vi "Riccati_Check_Detectable.vi"(9 "Q":T1, 11 "A":T1) -> (0 "error out":errorcluster, 1 "Stable Bad":bool, 2 "Pos Semi Definite":bool, 3 "Bad":bool, 4 "Q_Check":T1, 5 "C":T1, 6 "Q_Chk_Passed":bool)   [LabVIEW 2019, in "Trajectory_Library.lvlib"]
doc: "This function is for internal use, by the riccati_iput_check, ONLY.\n\nThis function check if (A,C) is a detectable pair, where Q = C' * C. (A,C) is detectable if and only if the unobservable eigenvalues of A, if any, have absolute values less than one, where an eigenvalue is unobservable if Rank[lambda * I - A; C] < n. Also, (A,C) is detectable if and only if (A',C') is stabilizable.\n\nInputs:\n - A -- A matrix\n - Q -- Q matrix\n\nOutputs:\n - Bad -- Returns TRUE, if the A,Q pair is not detectable or an error occured.\n - Error -- Error cluster that returns an error if A, Q is not detectable or some other error occured."
uses:
  Trajectory_Library.lvlib
  <vilib>/Analysis/Matrix/Datatypes/RealMatrix.ctl
  <vilib>/Analysis/_algsub.llb/Matrix Type for Test.ctl
  <vilib>/Analysis/baseanly.llb/Real A x B.vi
  <vilib>/Analysis/7linalg.llb/Real LU Factorization.vi
  <vilib>/Analysis/Matrix/Numeric/Subtract/Subtract - RM,RM.vi
  <vilib>/Analysis/Matrix/Numeric/Absolute Value/Absolute Value - RM.vi
  <vilib>/Analysis/_algsub.llb/Test Real Matrix Type.vi
  <vilib>/Analysis/NI_AALBase.lvlib
  <vilib>/Analysis/NI_AALPro.lvlib
  <vilib>/Analysis/Matrix/NI_Matrix.lvlib
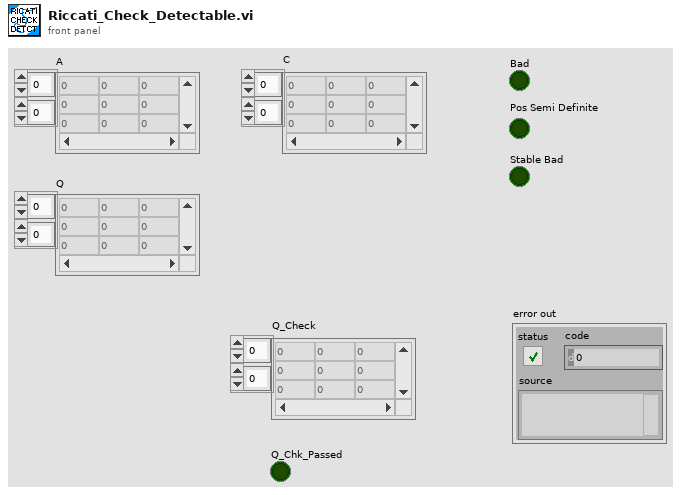
[diagram p1: front panel]
types:
  T1 = typedef "NI_Matrix.lvlib/RealMatrix.ctl" = dbl[][]
  T2 = typedef "NI_AALPro.lvlib/Matrix Type for Test.ctl" = i32
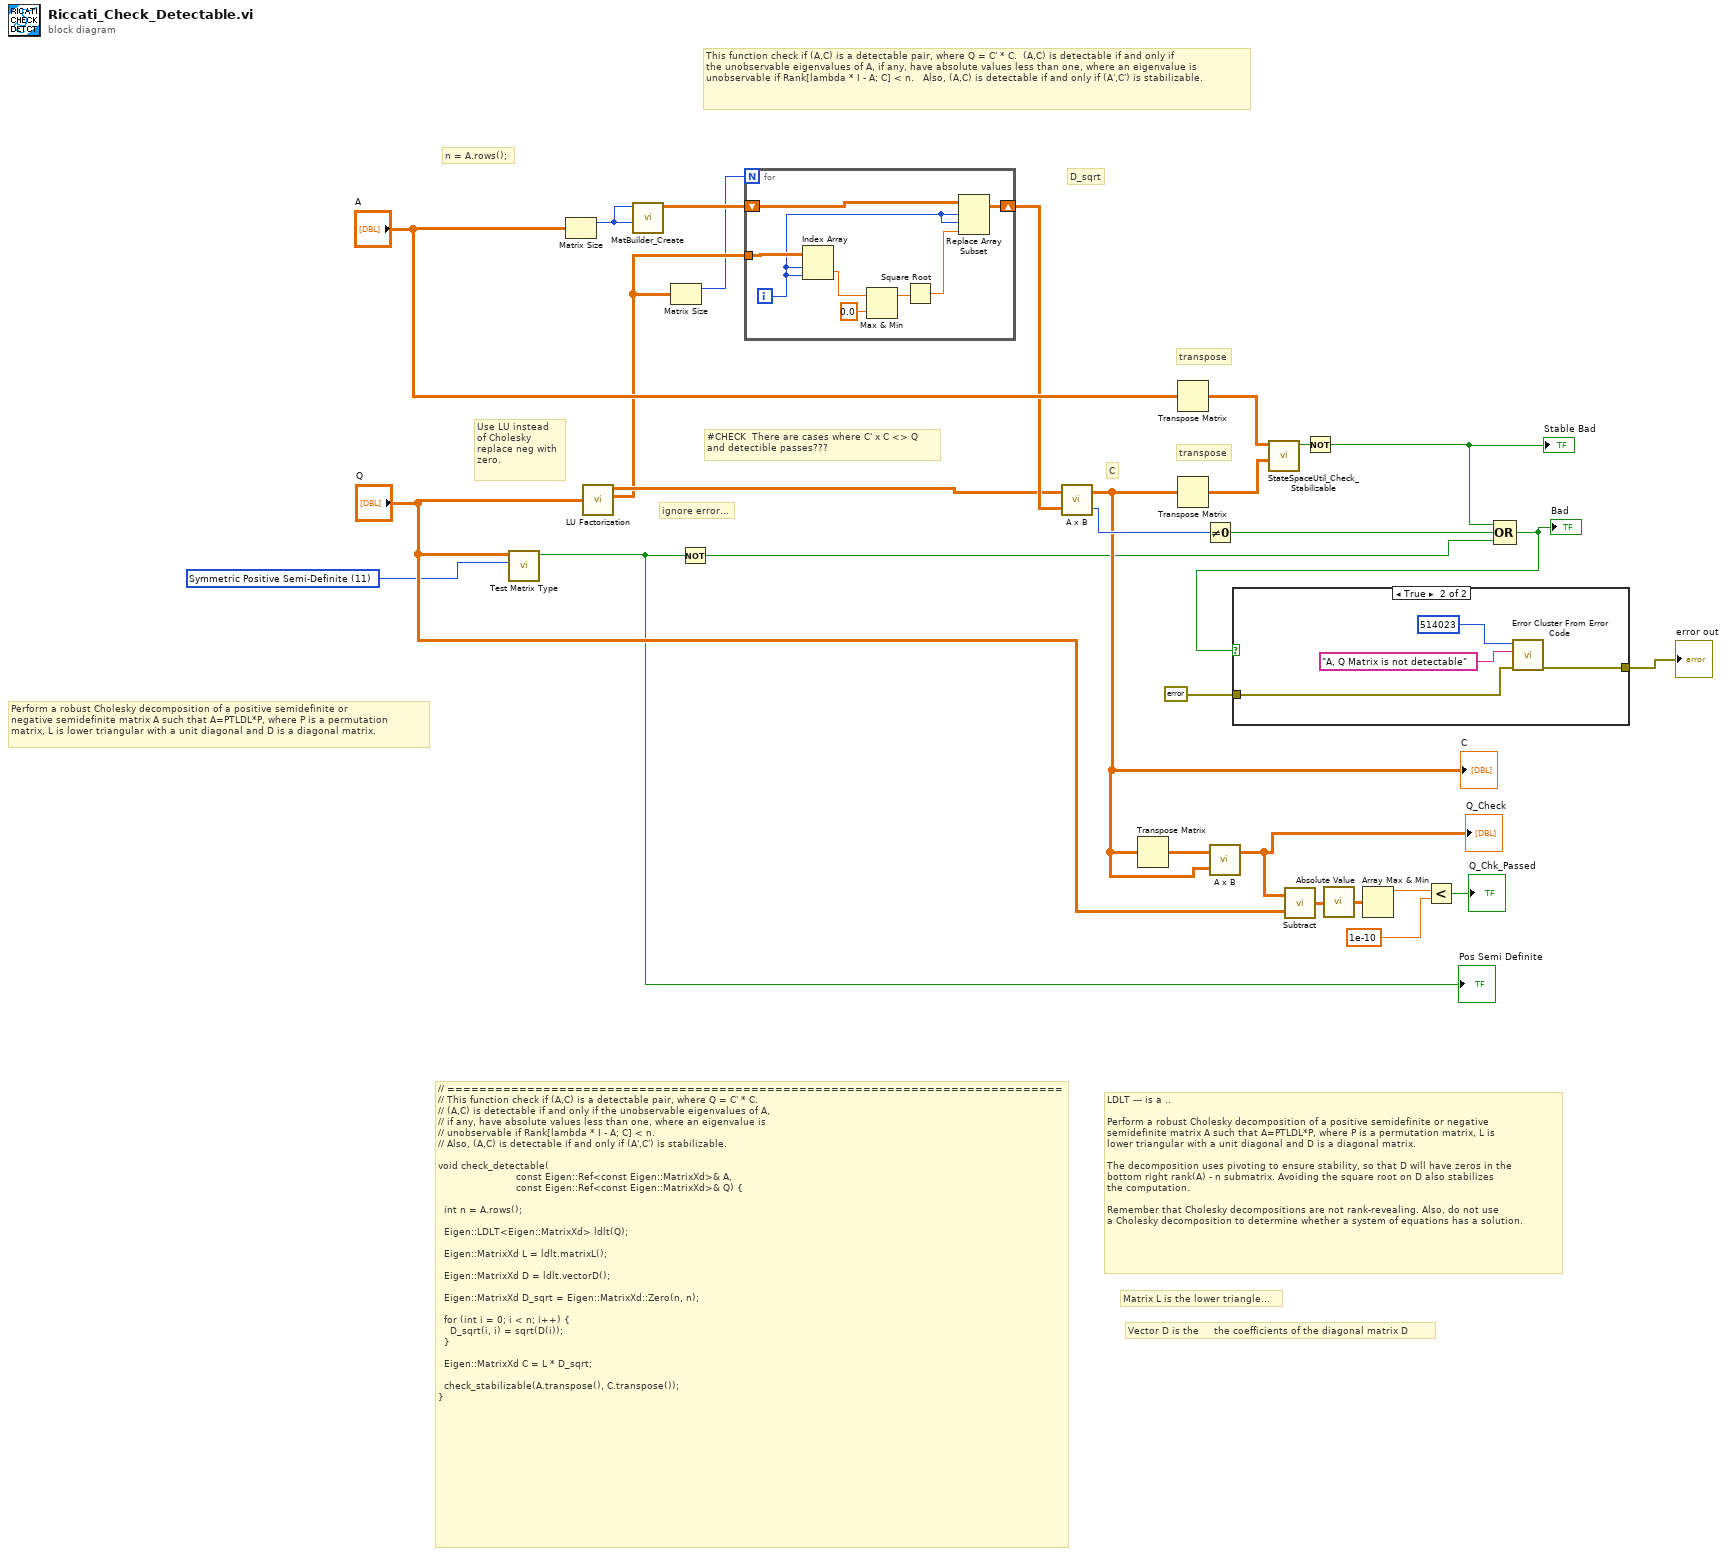
[diagram p0: block diagram]
diagram:
  w6 = T2 11 items=["Symmetric Positive Definite"=10, "Symmetric Positive Semi-Definite"=11, "Symmetric"=20, "Hermitian"=21] ("matrix type")
  # "#CHECK  There are cases where C' x C <> Q \nand detectible passes???"
  # "ignore error..."
  # "Use LU instead\nof Cholesky\nreplace neg with\nzero."
  # "C"
  # "Vector D is the     the coefficients of the diagonal matrix D"
  # "Matrix L is the lower triangle..."
  # "LDLT --- is a ..\n\nPerform a robust Cholesky decomposition of a positive semidefinite or negative \nsemidefinite matrix A such that A=PTLDL*P, where P is a permutation matrix, L is \nlower triangular with a unit diagonal and D is a diagonal matrix.\n\nThe decomposition uses pivoting to ensure stability, so that D will have zeros in the \nbottom right rank(A) - n submatrix. Avoiding the square root on D also stabilizes \nthe computation.\n\nRemember that Cholesky decompositions are not rank-revealing. Also, do not use \na Cholesky decomposition to determine whether a system of equations has a solution."
  # "This function check if (A,C) is a detectable pair, where Q = C' * C.  (A,C) is detectable if and only if \nthe unobservable eigenvalues of A, if any, have absolute values less than one, where an eigenvalue is \nunobservable if Rank[lambda * I - A; C] < n.   Also, (A,C) is detectable if and only if (A',C') is stabilizable."
  # "transpose"
  # "transpose"
  # "D_sqrt"
  # "Perform a robust Cholesky decomposition of a positive semidefinite or \nnegative semidefinite matrix A such that A=PTLDL*P, where P is a permutation \nmatrix, L is lower triangular with a unit diagonal and D is a diagonal matrix."
  # "n = A.rows();"
  # "// =============================================================================\n// This function check if (A,C) is a detectable pair, where Q = C' * C.\n// (A,C) is detectable if and only if the unobservable eigenvalues of A,\n// if any, have absolute values less than one, where an eigenvalue is\n// unobservable if Rank[lambda * I - A; C] < n.\n// Also, (A,C) is detectable if and only if (A',C') is stabilizable.\n\nvoid check_detectable(\n                          const Eigen::Ref<const Eigen::MatrixXd>& A,\n                          const Eigen::Ref<const Eigen::MatrixXd>& Q) {\n\n  int n = A.rows();\n\n  Eigen::LDLT<Eigen::MatrixXd> ldlt(Q);\n\n  Eigen::MatrixXd L = ldlt.matrixL();\n\n  Eigen::MatrixXd D = ldlt.vectorD();\n\n  Eigen::MatrixXd D_sqrt = Eigen::MatrixXd::Zero(n, n);\n\n  for (int i = 0; i < n; i++) {\n    D_sqrt(i, i) = sqrt(D(i));\n  }\n\n  Eigen::MatrixXd C = L * D_sqrt;\n\n  check_stabilizable(A.transpose(), C.transpose());\n}"
  n1 = call-poly <vilib>:"Test Matrix Type.vi"("matrix type"=w6, "Input Matrix"="Q") -> ("is type?"=w5:bool)  [unwired: 8 in, 1 out]
  "Pos Semi Definite" <- w5
  n2 = Matrix Size(0:"A") -> (1:w25:i32)  [unwired: 1 out]
  n3 = call-poly <vilib>:"LU Factorization.vi"("A"="Q") -> ("L"=w18:T1, "U"=w17:T1)  [unwired: 2 out]
  n4 = call "MatBuilder_Create.vi"("Columns"=w25, "Rows"=w25) -> ("output matrix"=w24:T1)  [unwired: 9 in]
  n5 = Matrix Size(0:w17) -> (1:w16:i32)  [unwired: 1 out]
  n6 = Not(x=w5) -> (.not. x?=w4:bool)
  n7 = for {
    N: w16 -> [_]
    tunnel: w17 -> [w36]
    shift-right: [w34] -> w22
    shift-left: w24 -> [w35]
    i -> [w29]
    n8 = Index Array(array=w36, index (row)=w29, index (col)=w29) -> (element=w32:dbl)
    n9 = Max & Min(x=w32, y=0.0) -> (max(x,y)=w30:dbl)  [unwired: 1 out]
    n10 = Square Root ("Square Root.vi")(x=w30) -> (sqrt(x)=w33:dbl)
    n11 = Replace Array Subset(array=w35, new element=w33, index (row)=w29, index (col)=w29) -> (w34:T1)
  }
  n12 = call-poly <vilib>:"A x B.vi"("B"=w22, "A"=w18) -> ("error"=w23:i32, "A x B"=w14:T1)
  "C" <- w14
  n13 = Transpose Matrix(1:w14) -> (0:w15:T1)
  n14 = Transpose Matrix(1:"A") -> (0:w28:T1)
  n15 = Transpose Matrix(1:w14) -> (0:w27:T1)
  n16 = Not Equal To 0?(x=w23) -> (x != 0?=w21:bool)
  n17 = call-poly <vilib>:"A x B.vi"("B"=w14, "A"=w15) -> ("A x B"=w13:T1)  [unwired: 1 out]
  "Q_Check" <- w13
  n18 = call "StateSpaceUtil_Check_Stabilizable.vi"("B"=w27, "A"=w28) -> ("IsStabilizable"=w20:bool)  [unwired: 6 in, 3 out]
  n19 = call-poly <vilib>:"Subtract.vi"("Real Matrix B"="Q", "Real Matrix A"=w13) -> ("A - B"=w12:T1)
  n20 = Not(x=w20) -> (.not. x?=w19:bool)
  "Stable Bad" <- w19
  n21 = call-poly <vilib>:"Absolute Value.vi"("Real Matrix A"=w12) -> ("|A|"=w11:T1)
  n22 = Array Max & Min(array=w11) -> (max value=w10:dbl)  [unwired: 3 out]
  n23 = Less?(x=w10, y=1e-10) -> (x < y?=→"Q_Chk_Passed":bool)
  n24 = Compound Arithmetic op=OR(w19, w21, w4) -> (w3:bool)
  "Bad" <- w3
  n25 = case shown="True" w3 {
    tunnel: errorcluster {"status"=FALSE, "code"=0, "source"=""} ("error constant") -> [w37 w39]
    tunnel: [w37 w38] -> w1
    frame False {
    }
    frame True {
      n26 = call <vilib>:"Error Cluster From Error Code.vi"("error in (no error)"=w39, "error message (\"\")"="A, Q Matrix is not detectable" ("error message (\"\")"), "error code (0)"=514023) -> ("error out"=w38:errorcluster)  [unwired: 6 in]
    }
  }
  "error out" <- w1
